vi "Log_write.vi"(8 "日志内容in 2":string, 9 "日志选择":string, 10 "日志内容in":string[](array[string]), 11 "创建的日志":string[](array[string])) -> (2 "日志内容out":string[](array[string]))   [LabVIEW 2018, in "Log_class.lvlib"]
uses:
  Log_class.lvlib
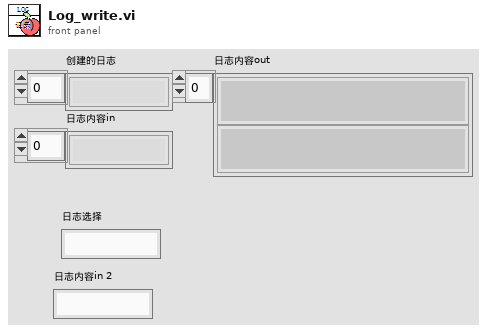
[diagram p1: front panel]
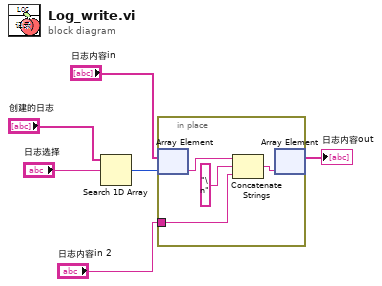
[diagram p0: block diagram]
diagram:
  n1 = Search 1D Array(1D array="创建的日志", element="日志选择") -> (index of element=w6:i32)  [unwired: 1 in]
  n2 = in-place {
    in-place-border: "日志内容in 2" -> [w7]
    n3 = in-place-array #1("日志内容in", w6) -> (w10:string)
    n4 = Concatenate Strings(w10, "\n" ("字符串"), w7) -> (w8:string)
    n5 = in-place-array #1(w8) -> (→"日志内容out":string[])  [unwired: 1 out]
  }
